vi "Run Test - Calc T50 T90 T100 (SubVI) (1).vi"(4 "Test Stage":string, 6 "fileid":string, 8 "error in (no error)":errorcluster, 10 "Enum":T1, 11 "Cluster in":T2 {"M Event" items=["Stop", "Running", "PID", "Up Limit", "Down Limit", "Load Limit"]; "Test Type" items=["Please Select", "Triaxial Shear", "Triaxial UU", "Shearbox", "Permeability", "Consolidation (Stepped Loading)/Swelling", "Saturation (Incremental)", "User Defined", "UCT", "Isotropic Consolidation", "Swelling Pressure", "B-Check", "Saturation (Step Increment)", "Saturation (Ramp)"]; "Data"."Test Type" items=["Please Select", "Triaxial Shear", "Triaxial UU", "Shearbox", "Permeability", "Consolidation (Stepped Loading)/Swelling", "Saturation (Incremental)", "User Defined", "UCT", "Isotropic Consolidation", "Swelling Pressure", "B-Check", "Saturation (Step Increment)", "Saturation (Ramp)"]}) -> (0 "error out":errorcluster, 3 "Cluster out":T2 {"M Event" items=["Stop", "Running", "PID", "Up Limit", "Down Limit", "Load Limit"]; "Test Type" items=["Please Select", "Triaxial Shear", "Triaxial UU", "Shearbox", "Permeability", "Consolidation (Stepped Loading)/Swelling", "Saturation (Incremental)", "User Defined", "UCT", "Isotropic Consolidation", "Swelling Pressure", "B-Check", "Saturation (Step Increment)", "Saturation (Ramp)"]; "Data"."Test Type" items=["Please Select", "Triaxial Shear", "Triaxial UU", "Shearbox", "Permeability", "Consolidation (Stepped Loading)/Swelling", "Saturation (Incremental)", "User Defined", "UCT", "Isotropic Consolidation", "Swelling Pressure", "B-Check", "Saturation (Step Increment)", "Saturation (Ramp)"]})   [LabVIEW 2019]
uses:
  Controls/RunTest - Data Structure.ctl
  Controls/Test Panel - Data Structure.ctl
  Controls/Station - Test Type.ctl
  <vilib>/Utility/miscctls.llb/LVRowAndColumnTypeDef.ctl
  Controls/RunTest - Calculate Data.ctl
  <vilib>/httpClient/ClientHandle.ctl
  Controls/RunTest - Start Condition.ctl
  Controls/RunTest - Stop Condition.ctl
  Controls/UDP - Event.ctl
  Controls/RunTest - State.ctl
  Controls/eFGV States.ctl
  <vilib>/httpClient/LabVIEWHTTPClient.lvlib
types:
  T1 = typedef "RunTest - State.ctl" = enum16{"Load Testfile", "Notifier", "Init", "Idle", "Load", "Read DB", "Run", "Pause", "Stop", "Check Start", "Check Stop", "Check Post Stop", "Check Log", "EndStage", "Data View", "Data View PWP", "Display", "Graph", "Graph PWP", "Close", "Stop PID", "Check Limit", "Auto", "Up", "Log", "Zero", "Machine Control", "Save Report"}
  T2 = typedef "RunTest - Data Structure.ctl" = cluster{"Test Plan":string[], "PlanRow":i32, "Device Name":string[], "Timeout":i32, "Start?":bool, "Pause?":bool, "IP Address":string[], "LogRow":i32, "Logtype":u16, "Log Elapse":sgl, "Data":T3, "Stop log?":bool, "tdms":refnum<k34>, "Sensor Data":sgl[], "Start time":timestamp, "Prev Log Elapse":u32, "Plot":u16, "X-Axis":u16[], "Y-Axis":u16[], "XY":cluster{"X":dbl, "Y":dbl}[][], "End Stage?":bool, "1run":bool, "Condition":u16[], "Start Con":bool, "Log Con":bool, "Stop Con":bool, "Start Elapse":dbl, "Start Load":dbl, "Motor":i32, "StartRow":i32, "number log":i32, "Dir":bool, "Start time test":timestamp, "Auto":bool, "Check return?":bool, "Inv":cluster{"M":i32[], "Bool":bool[]}, "tdms temp":refnum<k34>, "Zero?":bool, "Plot Timer":dbl, "1st Run":bool, "TDMS Path":path, "MaxLoad":dbl, "Log Timer":sgl[], "Test Type":T4, "Log Sensor":string[], "Save?":bool, "1st Log":bool, "Y-Axis 2":u16[], "On Y-Axis 2":bool, "Decimal":u8[], "Init":cluster{"PWP TS":sgl, "Load TS":sgl, "Volume TS":sgl, "Disp TS":sgl, "CP":sgl, "Vol In":sgl, "Vol Out":sgl, "Load UCT":sgl, "Disp UCT":sgl, "PWP Sat":sgl, "CP Sat":sgl, "Volume IsoCons":sgl, "PWP IsoCons":sgl, "PWP TUU":sgl, "Load TUU":sgl, "Volume TUU":sgl, "Disp TUU":sgl, "Load Cons":sgl, "Disp Cons":sgl, "Volume Sat":sgl, "Vertical Load SB":sgl, "Vertical Disp SB":sgl, "H Disp SB":sgl, "H Load SB":sgl, "PWP BC":sgl, "CP BC":sgl, "PWP Sat Step":sgl, "CP Sat Step":sgl, "Volume Sat Step":sgl, "PWP Sat Ramp":sgl, "CP Sat Ramp":sgl, "Volume Sat Ramp":sgl}, "Calc":T6, "Device Index":i32[], "Channel Index":i32[], "http ref":T7, "fileid":string, "Step Cons":cluster{"V Stress":sgl, "H Settlement":sgl}, "RunTest":bool, "Graph Last":i32, "Init?":bool, "Datalog":bool[], "Start":T8, "Stop":T9, "Running?":bool, "StartTime":dbl, "Log Prev Time":dbl, "KeyName":string[], "Test RunTime":dbl, "Log Prev Axial":dbl, "M Event":T10[], "Last Log":bool, "popup":bool, "PreStart UU":bool, "PreStart Sat":bool, "PreStart BC":bool, "PreStart Sat Step":bool, "PreStart Sat Ramp":bool, "Prev Sat IP":string}
  T3 = typedef "Test Panel - Data Structure.ctl" = cluster{"Station":string, "Sample ID":string, "Job No":string, "Job Description":string, "Filename":string, "Test Type":T4, "Speciment No":string, "Depth":string, "Height":string, "Diameter/Length":string, "Weight":string, "Test Parameter":string, "Station[]":string[], "Edit Pos":T5, "Edit Pos Prev":T5, "Area":string, "Path":string, "sample_id":string}
  T4 = typedef "Station - Test Type.ctl" = u16
  T5 = typedef "LVRowAndColumnTypeDef.ctl" = cluster{"Row":i32, "Column":i32}
  T6 = typedef "RunTest - Calculate Data.ctl" = cluster{"TS":cluster{"Change PWP":sgl, "Change Vol":sgl, "Axial Load":sgl, "CiL":sgl, "Deviator":sgl, "Axial Strain":sgl, "MaxDeviator":sgl, "SS":sgl, "CAS":sgl}, "TUU":cluster{"Change PWP":sgl, "Axial Load":sgl, "CiL":sgl, "Deviator":sgl, "Axial Strain":sgl, "MaxDeviator":sgl}, "Sat":cluster{"B Value":sgl, "PWP Diss":sgl, "CPP":sgl, "CV":sgl}, "Per":cluster{"Change Vol In":sgl, "Change Vol Out":sgl, "Mean Vol":sgl, "Gradient Pressure":sgl, "Outlet Flow":sgl, "Inlet Flow":sgl, "I X1":sgl, "I X2":sgl, "I Y1":sgl, "I Y2":sgl, "O X1":sgl, "O X2":sgl, "O Y1":sgl, "O Y2":sgl}, "Step Cons":cluster{"V Stress":sgl, "H Settlement":sgl, "Total H Settle":sgl, "Prev Total H":sgl}, "UCT":cluster{"ALC":sgl, "H Change":sgl, "Deviator":sgl, "Axial Strain":sgl, "V Stress":sgl, "MaxDeviator":sgl}, "ISO Cons":cluster{"CPP":sgl, "PWP Diss":sgl, "CV":sgl, "VS":sgl}, "SB":cluster{"Speci LenC":sgl, "Shear Strain":sgl, "H LC":sgl, "Normal Stress":sgl, "Shear Stress":sgl, "MaxShear":sgl}, "BC":cluster{"B Value":sgl, "PWP Diss":sgl, "CPP":sgl, "CV":sgl}, "Sat Step":cluster{"B Value":sgl, "PWP Diss":sgl, "CPP":sgl, "CV":sgl}, "Sat Ramp":cluster{"B Value":sgl, "PWP Diss":sgl, "CPP":sgl, "CV":sgl}, "Prev Log":string[]}
  T7 = typedef "LabVIEWHTTPClient.lvlib/ClientHandle.ctl" = refnum<k1>
  T8 = typedef "RunTest - Start Condition.ctl" = cluster{"Cons":cluster{"VS":dbl, "Delay":bool, "No Delay":dbl}, "Sat":cluster{"CP":dbl, "BP":dbl, "StartBP":bool, "Target CP":bool, "Target BP":bool}, "Iso":cluster{"Select":dbl, "BP":dbl, "IC2":dbl, "IC3":dbl, "IC4":dbl, ". IC6":bool, "IC6":dbl, "IC6-2":dbl, "Time Cond":dbl, "Last PWP":dbl, "Target CP":bool, "Target BP":bool, "NewCP":dbl, "NewBP":dbl, "Noti CP":bool, "Noti BP":bool, "Noti PWP":bool, "PrevSatBP":dbl}, "TS":cluster{"SS":dbl, "Engage":bool, "ES":dbl, "LC":dbl, "PreStart":bool, "Trig SS":bool, "Drain":dbl, "Select":u16, "Max SS .":bool, "MaxSS":dbl}, "TUU":cluster{"SS":dbl, "Engage":bool, "ES":dbl, "LC":dbl, "PreStart":bool, "Trig SS":bool, "CP":dbl, "Delay Value":dbl, "Delay":bool, "CP PID":bool}, "UCT":cluster{"SS":dbl, "Engage":bool, "ES":dbl, "LC":dbl, "PreStart":bool, "Trig SS":bool}, "Enable?":bool, "SB":cluster{"SS":dbl, "Engage":bool, "ES":dbl, "LC":dbl, "PreStart":bool, "Trig SS":bool, "VS":dbl, "Delay Value":dbl, "Delay":bool, "VS PID":bool}, "Perm":cluster{"DP":dbl}, "BC":cluster{"CP":dbl, "Target CP":bool, "Target BP":bool, "CP Inc":dbl, "CP .Init":bool, "CP Init":dbl, "1st BC":bool}, "Sat (Step)":cluster{"Select":dbl, "CP":dbl, "BP":dbl, "EP":dbl, "StartCP":bool, "Target CP":bool, "Target BP":bool}, "Sat (Ramp)":cluster{"Select":dbl, "CP":dbl, "BP":dbl, "EP":dbl, "StartCP":bool, "Target CP":bool, "Target BP":bool, "Time Rate":u32}}
  T9 = typedef "RunTest - Stop Condition.ctl" = cluster{"Cons":cluster{"Select":i32, "Disp":dbl, "Time":dbl, "Time2":dbl, "Disp 2":dbl, "Time Cond":dbl, "Last Disp":dbl, "Swell":bool, "T50,90,100":cluster{"t50_x_min":dbl, "t50_y_value":dbl, "t90_x_min":dbl, "t90_y_value":dbl, "t100_x_min":dbl, "t100_y_value":dbl, "target_column":string, "test_type":string, "error":string}}, "Sat":cluster{"Select":i32, "PP":dbl, "Time":dbl, "VC":dbl, "Time2":dbl, "Time Cond":dbl, "Last PP":dbl, ".B":bool, "B":dbl, "Last Vc":dbl, "Time Cond 2":dbl, "Time3":dbl, "Time Cond 3":dbl, "B Achieve":bool, "PP Achieve":bool, "VC Achieve":bool, "Max Achieve":bool, "CP Check":dbl, "Skip Next":bool, "B Achieve Stage":u32, ".CP Check":bool}, "Iso":cluster{"PP":dbl, "Time":dbl, "VC":dbl, "Time2":dbl, "Time Cond":dbl, "Last Vc":dbl, ".PP":bool, "Time Cond 2":dbl, "Select":i32, "BS":cluster{"t50_x_min":dbl, "t50_y_value":dbl, "t90_x_min":dbl, "t90_y_value":dbl, "t100_x_min":dbl, "t100_y_value":dbl, "target_column":string, "test_type":string, "error":string}, "Final VC":dbl, "ASTM":cluster{"t50_x_min":dbl, "t50_y_value":dbl, "t90_x_min":dbl, "t90_y_value":dbl, "t100_x_min":dbl, "t100_y_value":dbl, "target_column":string, "test_type":string, "error":string}, "ASTM Log":cluster{"t50_x_min":dbl, "t50_y_value":dbl, "t90_x_min":dbl, "t90_y_value":dbl, "t100_x_min":dbl, "t100_y_value":dbl, "target_column":string, "test_type":string, "error":string}, "PP Achieve":bool, "VC Achieve":bool}, "TS":cluster{"Axial":dbl, ".MaxDev":bool, "MaxDev Value":dbl, "Return":bool, "Reset":bool, "Prev Time":dbl, "PostStop Run":bool, "CP Stop":bool, "BP Stop":bool, "PostStop Trig":bool, "Reset Value":dbl, "BPTrig":bool, "CPTrig":bool, "VLCTrig":bool, "CAxial":dbl, "Select":i32}, "TUU":cluster{"Axial":dbl, ".MaxDev":bool, "MaxDev Value":dbl, "Return":bool, "Reset":bool, "Prev Time":dbl, "PostStop Run":bool, "CP Stop":bool, "BP Stop":bool, "PostStop Trig":bool, "Reset Value":dbl, "BPTrig":bool, "CPTrig":bool, "VLCTrig":bool}, "UCT":cluster{"Axial":dbl, ".MaxDev":bool, "MaxDev Value":dbl, "Return":bool, "Reset":bool, "Prev Time":dbl, "PostStop Run":bool, "CP Stop":bool, "BP Stop":bool, "PostStop Trig":bool}, "Enable?":bool, "SB":cluster{"Shear":dbl, ".MaxShear":bool, "MaxShear Value":dbl, "Return":bool, "Reset":bool, "Prev Time":dbl, "PostStop Run":bool, "CP Stop":bool, "BP Stop":bool, "PostStop Trig":bool, "Reset Value":dbl, "BPTrig":bool, "CPTrig":bool, "VLCTrig":bool}, "Perm":cluster{"Max Time":bool, "Reset":bool, "PostStop Run":bool, "Ratio":bool, "Reset Value":dbl, "Time":dbl, "RatioTime":dbl, "RatioMore":dbl, "RatioLess":dbl, "Time Cond":dbl, "Time Cond 2":dbl, "Prev IF":dbl, "Prev OF":dbl, "PostStop Trig":bool, "BP Trig":bool, "DP Stop":bool, "BP Stop":bool, "CP Stop":bool, "CP Trig":bool}, "SP":cluster{".Max Time":bool, ".Time":bool, "Time":dbl, "MaxTime":dbl, "Time Cond":dbl, "Max Time Cond":dbl, "Stress":dbl}, "BC":cluster{"Select":i32, "PP":dbl, "Time":dbl, "Time Cond":dbl, "Last PP":dbl, ".B":bool, "B":dbl, "Time 2":dbl, "Time Cond 2":dbl, "B Achieve":bool, "PP Achieve":bool, "Max Achieve":bool, "CP Check":dbl, "Skip Next":bool, "B Achieve Stage":u32, ".CP Check":bool}, "Sat (Step)":cluster{"Select":i32, "PP":dbl, "Time":dbl, "VC":dbl, "Time2":dbl, "Time Cond":dbl, "Last PP":dbl, ".B":bool, "B":dbl, "Last Vc":dbl, "Time Cond 2":dbl, "Time3":dbl, "Time Cond 3":dbl, "B Achieve":bool, "PP Achieve":bool, "VC Achieve":bool, "Max Achieve":bool, "CP Check":dbl, "Skip Next":bool, "B Achieve Stage":u32}, "Sat (Ramp)":cluster{"Select":i32, "PP":dbl, "Time":dbl, "VC":dbl, "Time2":dbl, "Time Cond":dbl, "Last PP":dbl, ".B":bool, "B":dbl, "Last Vc":dbl, "Time Cond 2":dbl, "Time3":dbl, "Time Cond 3":dbl, "B Achieve":bool, "PP Achieve":bool, "VC Achieve":bool, "Max Achieve":bool, "CP Check":dbl, "Skip Next":bool, "B Achieve Stage":u32}}
  T10 = typedef "UDP - Event.ctl" = u16
  T11 = cluster{"t50_x_minutes":dbl, "t50_y_value":dbl, "t90_x_minutes":dbl, "t90_y_value":dbl, "t100_x_minutes":dbl, "t100_y_value":dbl, "target_column":string, "test_type":string, "error":string}
  T12 = typedef "eFGV States.ctl" = enum16{"Init", "Read", "Write", "Exit"}
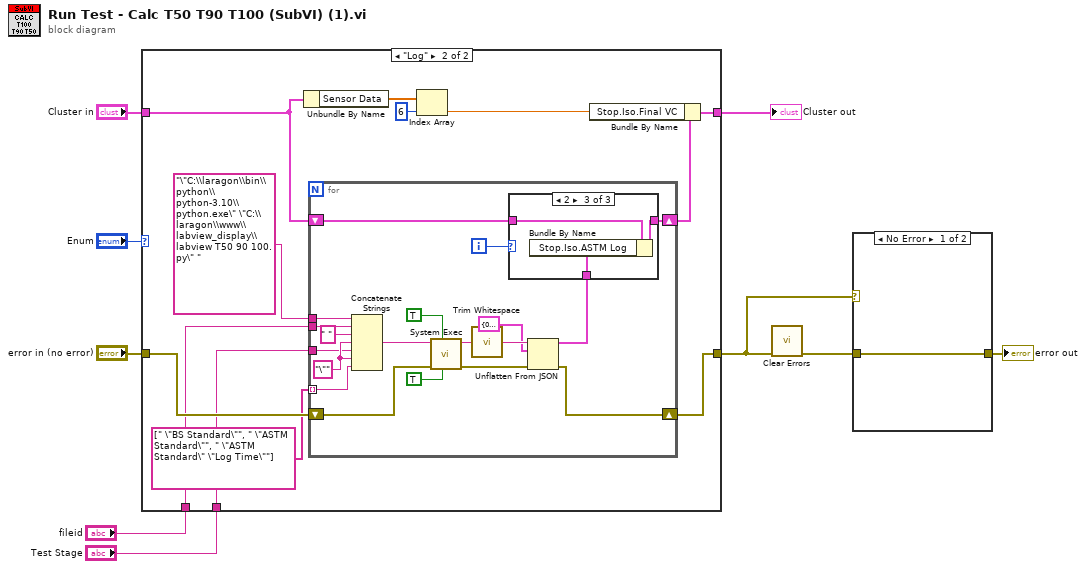
[diagram p0: block diagram]
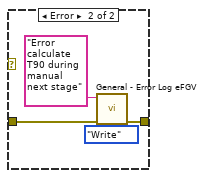
[diagram p2: hidden frame]
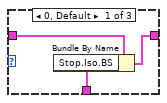
[diagram p4: hidden frame]
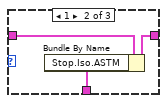
[diagram p5: hidden frame]
diagram:
  n1 = case shown="\"Log\"" "Enum" {
    tunnel: "error in (no error)" -> [w11 w22]
    tunnel: [w11 w21] -> w1
    tunnel: "Test Stage" -> [_ w20]
    tunnel: "fileid" -> [_ w19]
    tunnel: [w10 w18] -> w8
    tunnel: "Cluster in" -> [w10 w12]
    frame Default {
    }
    frame "Log" {
      n2 = Unbundle By Name(w12) -> ("Sensor Data"=w17:sgl[])
      n3 = for {
        tunnel: "\"C:\\laragon\\bin\\python\\python-3.10\\python.exe\" \"C:\\laragon\\www\\labview_display\\labview T50 90 100.py\" " ("command line") -> [w37]
        tunnel: w20 -> [w30]
        tunnel: w19 -> [w29]
        shift-right: [w31] -> w21
        shift-left: w22 -> [w32]
        tunnel: string[] [" \"BS Standard\"", " \"ASTM Standard\"", " \"ASTM Standard\" \"Log Time\""] -> [w26] mode=indexing
        shift-right: [w27] -> w13
        shift-left: w12 -> [w28]
        i -> [w25]
        w35 = "\"" ("string")
        n4 = Concatenate Strings(w37, w29, " " ("string"), w35, w30, w35, w26) -> (w39:string)
        n5 = call <vilib>:"System Exec.vi"("run minimized? (F)"=TRUE, "wait until completion? (T)"=TRUE, "error in (no error)"=w32, "command line"=w39) -> ("error out"=w42:errorcluster, "standard output"=w41:string)  [unwired: 4 in, 2 out]
        n6 = call <vilib>:"Trim Whitespace.vi"("string"=w41) -> ("trimmed string"=w40:string)  [unwired: 1 in]
        n7 = Unflatten From JSON(JSON string=w40, type and defaults=T11 {"t50_x_minutes"=0.0, "t50_y_value"=0.0, "t90_x_minutes"=0.0, "t90_y_value"=0.0, "t100_x_minutes"=0.0, "t100_y_value"=0.0, "target_column"="", "test_type"="", "error"=""}, error in (no error)=w42) -> (value=w24:T11, error out=w31:errorcluster)  [unwired: 4 in]
        n8 = case shown="2" w25 {
          tunnel: w28 -> [w45 w48 w51]
          tunnel: [w44 w47 w50] -> w27
          tunnel: w24 -> [w43 w46 w49]
          frame 0, Default {
            n9 = Bundle By Name(cluster=w45, "Stop.Iso.BS"=w43) -> (w44:T2)
          }
          frame 1 {
            n10 = Bundle By Name(cluster=w48, "Stop.Iso.ASTM"=w46) -> (w47:T2)
          }
          frame 2 {
            n11 = Bundle By Name(cluster=w51, "Stop.Iso.ASTM Log"=w49) -> (w50:T2)
          }
        }
      }
      n12 = Index Array(array=w17, index=6) -> (element=w15:sgl)
      n13 = Bundle By Name(cluster=w13, "Stop.Iso.Final VC"=w15) -> (w18:T2)
    }
  }
  "Cluster out" <- w8
  n14 = call <vilib>:"Clear Errors.vi"("error in (no error)"=w1) -> ("error out"=w3:errorcluster)  [unwired: 5 in, 1 out]
  n15 = case shown="No Error" w1 {
    tunnel: w3 -> [w52 w55]
    tunnel: [w52 w54] -> w2
    frame No Error {
    }
    frame Error {
      n16 = call "General - Error Log eFGV.vi"("eFGV States"=eFGV_States."Write", "error in (no error)"=w55, "Error In"="Error calculate T90 during manual next stage") -> ("error out"=w54:errorcluster)  [unwired: 6 in, 2 out]
    }
  }
  "error out" <- w2
